vi "Images.vi"() -> ()   [LabVIEW 2019]
uses:
  Classes/Parse/ParseXML/Path.ctl
  Classes/Parse/ParseXML/ParseSVG.lvclass
  Classes/Identity/Identifier.lvclass
  Classes/Identity/Associations.ctl
panel:
  out "String":string
  out "Array 9":string[][](array[string])
  out "Array 2":T1[](array[typedef])
  out "text":string
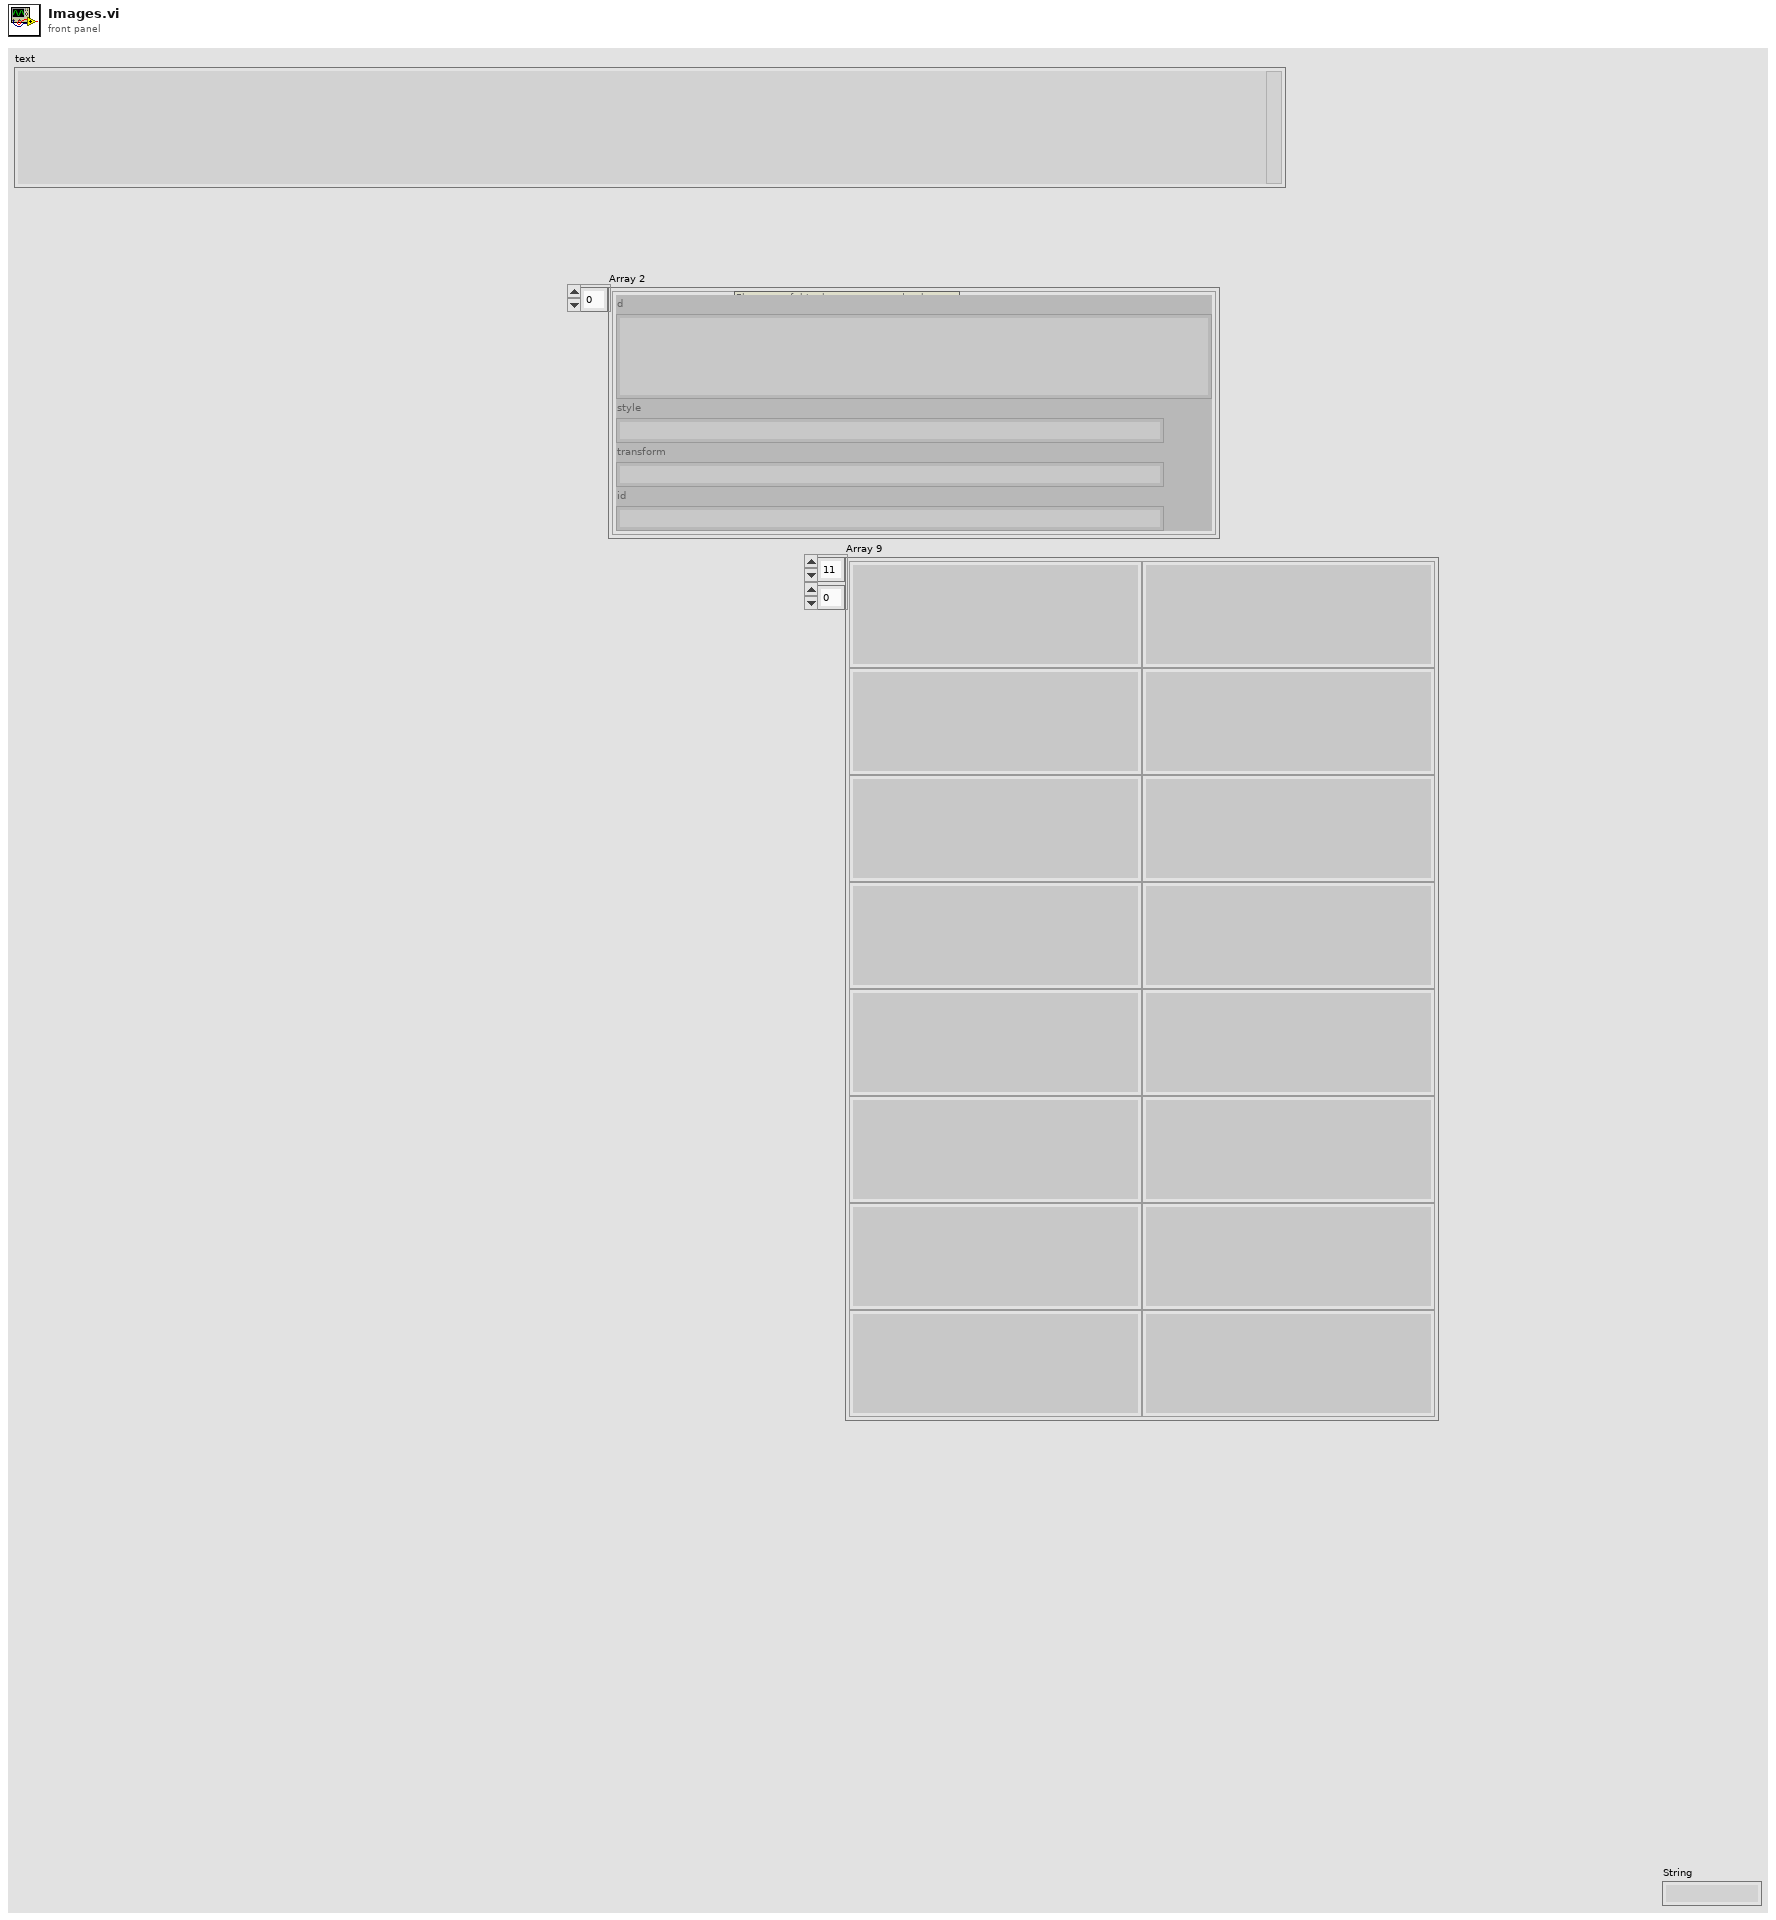
[diagram p1: front panel]
types:
  T1 = typedef "ParseSVG.lvclass/Path.ctl" = cluster{"d":string, "style":string, "transform":string, "id":string}
  T2 = typedef "Identifier.lvclass/Associations.ctl" = cluster{"Name":string, "Alias":string}
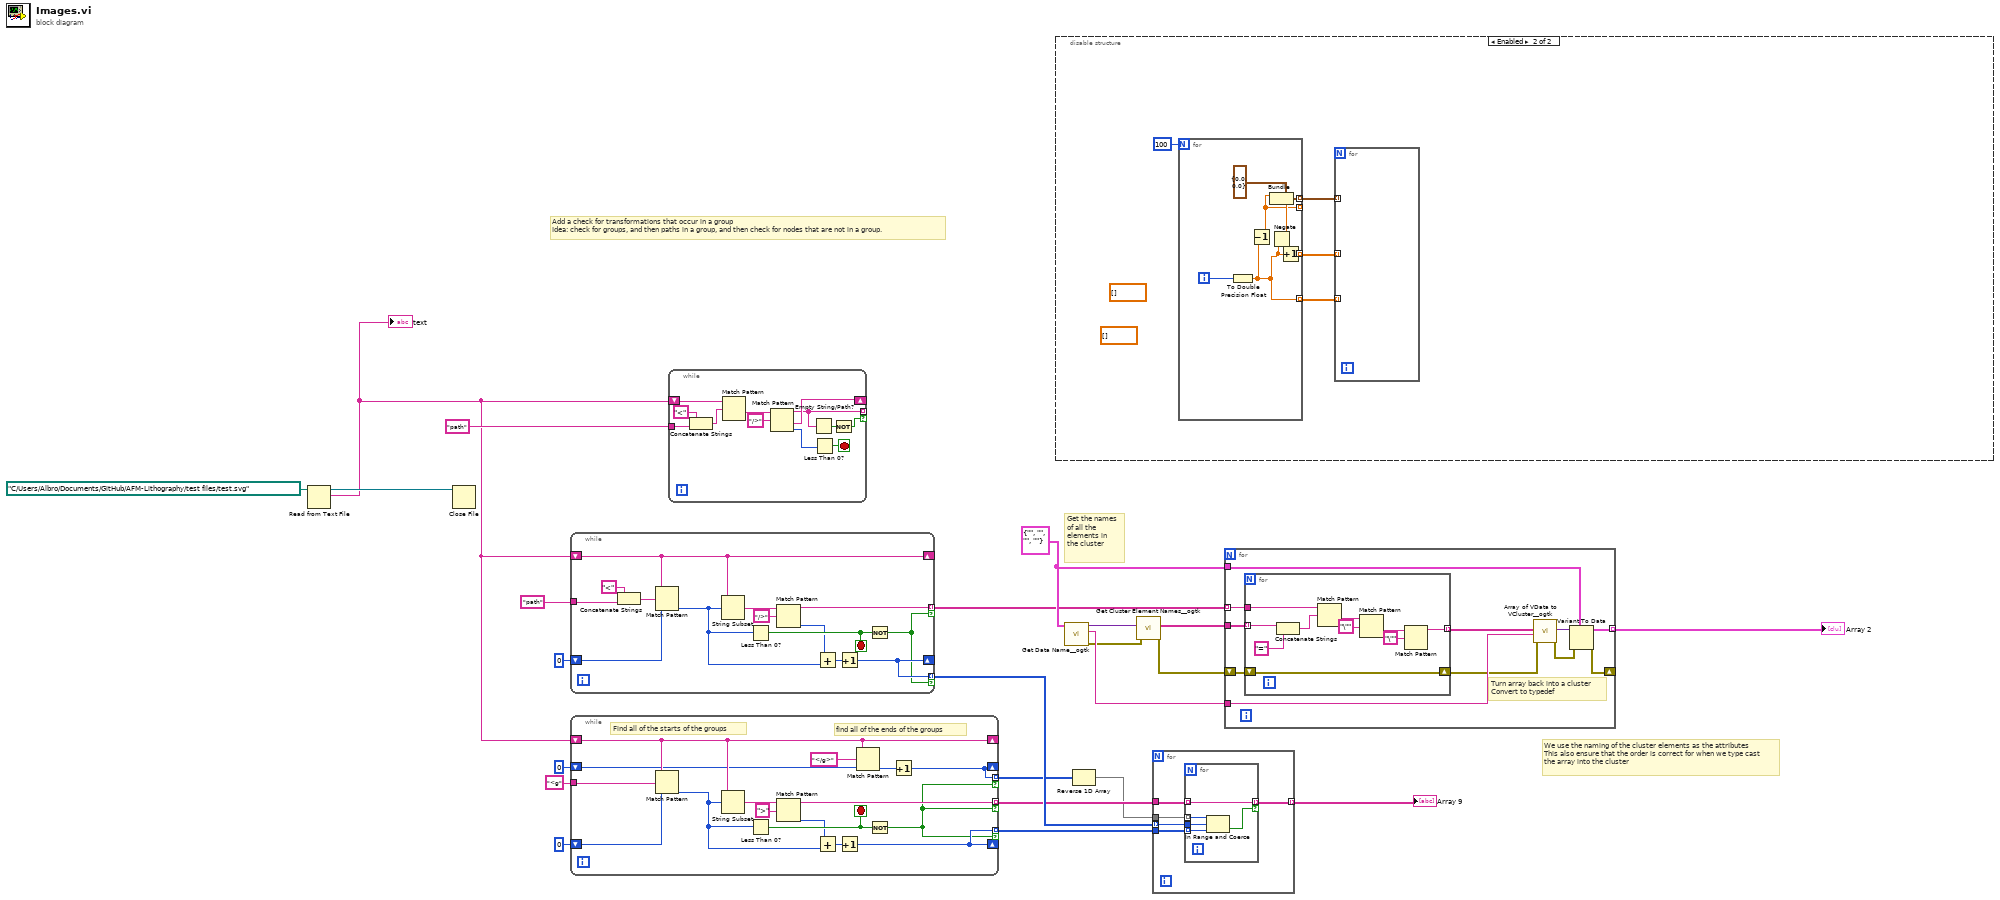
[diagram p0: block diagram]
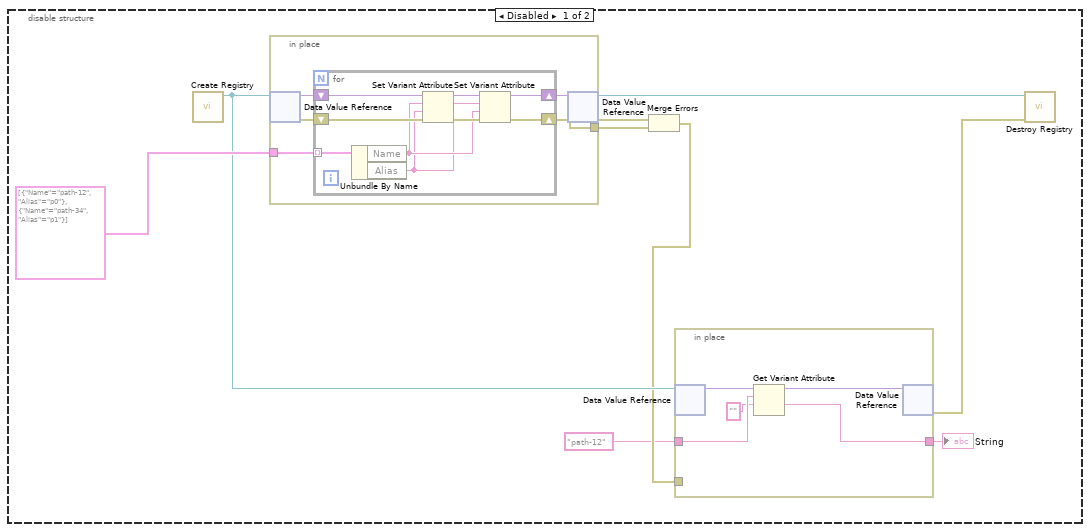
[diagram p2: hidden frame]
diagram:
  w15 = T1 {"d"="", "style"="", "transform"="", "id"=""} ("Path")
  # "Add a check for transformations that occur in a group\nIdea: check for groups, and then paths in a group, and then check for nodes that are not in a group."
  # "We use the naming of the cluster elements as the attributes\nThis also ensure that the order is correct for when we type cast the array into the cluster"
  # "Get the names of all the elements in the cluster"
  n1 = Read from Text File(file (use dialog)=path "C:/Users/Albro/Documents/GitHub/AFM-Lithography/test files/test.svg") -> (refnum out=w23:refnum<file>, text=w3:string)  [unwired: 3 in, 2 out]
  "text" <- w3
  n2 = Close File(refnum=w23) -> ()  [unwired: 1 in, 2 out]
  n3 = while {
    shift-right: [w37] -> _
    shift-left: w3 -> [w37]
    shift-right: [w25] -> _
    shift-left: 0 -> [w35]
    tunnel: [w32] -> w2 mode=indexing if=w24
    tunnel: "path" -> [w26]
    tunnel: [w25] -> w9 mode=indexing if=w24
    stop <- w31 stop-if-true
    n4 = Concatenate Strings("<" ("regular expression"), w26) -> (w28:string)
    n5 = Match Pattern(string=w37, regular expression=w28, offset (0)=w35) -> (offset past match=w29:i32)  [unwired: 3 out]
    n6 = String Subset(string=w37, offset (0)=w29) -> (substring=w36:string)  [unwired: 1 in]
    n7 = Less Than 0?(x=w29) -> (x < 0?=w31:bool)
    n8 = Match Pattern(string=w36, regular expression="/>") -> (before substring=w32:string, offset past match=w30:i32)  [unwired: 1 in, 2 out]
    n9 = Add(x=w30, y=w29) -> (x+y=w34:i32)
    n10 = Increment(x=w34) -> (x+1=w25:i32)
    n11 = Not(x=w31) -> (.not. x?=w24:bool)
  }
  n12 = while {
    shift-right: [w46] -> _
    shift-left: w3 -> [w46]
    shift-right: [w43] -> _
    shift-left: 0 -> [w52]
    tunnel: [w49] -> w7 mode=indexing if=w42
    tunnel: "<g" -> [w38]
    tunnel: [w39] -> w6 mode=indexing if=w42
    tunnel: [w43] -> w8 mode=indexing if=w42
    shift-right: [w39] -> _
    shift-left: 0 ("offset past match") -> [w41]
    stop <- w48 stop-if-true
    # "Find all of the starts of the groups"
    # "find all of the ends of the groups"
    n13 = Match Pattern(string=w46, regular expression=w38, offset (0)=w52) -> (offset past match=w44:i32)  [unwired: 3 out]
    n14 = String Subset(string=w46, offset (0)=w44) -> (substring=w53:string)  [unwired: 1 in]
    n15 = Less Than 0?(x=w44) -> (x < 0?=w48:bool)
    n16 = Match Pattern(string=w53, regular expression=">") -> (before substring=w49:string, offset past match=w47:i32)  [unwired: 1 in, 2 out]
    n17 = Add(x=w47, y=w44) -> (x+y=w51:i32)
    n18 = Increment(x=w51) -> (x+1=w43:i32)
    n19 = Match Pattern(string=w46, regular expression="</g>", offset (0)=w41) -> (offset past match=w40:i32)  [unwired: 3 out]
    n20 = Not(x=w48) -> (.not. x?=w42:bool)
    n21 = Increment(x=w40) -> (x+1=w39:i32)
  }
  n22 = while {
    shift-right: [w58] -> _
    shift-left: w3 -> [w65]
    tunnel: "path" -> [w64]
    tunnel: [w56] -> _ mode=indexing if=w57
    stop <- w60 stop-if-true
    n23 = Concatenate Strings("<" ("regular expression"), w64) -> (w63:string)
    n24 = Match Pattern(string=w65, regular expression=w63) -> (after substring=w62:string)  [unwired: 1 in, 3 out]
    n25 = Match Pattern(string=w62, regular expression="/>") -> (before substring=w56:string, after substring=w58:string, offset past match=w54:i32)  [unwired: 1 in, 1 out]
    n26 = Empty String/Path?(string/path=w56) -> (empty?=w59:bool)
    n27 = Less Than 0?(x=w54) -> (x < 0?=w60:bool)
    n28 = Not(x=w59) -> (.not. x?=w57:bool)
  }
  n29 = disable-structure shown="Enabled" {
    frame Disabled {
      n30 = call "Create Registry.vi"() -> ("Registry"=w70:refnum<data-value>)  [unwired: 10 in, 1 out]
      n31 = in-place {
        in-place-border: [w76] -> w71
        in-place-border: T2[] [{"Name"="path-12", "Alias"="p0"}, {"Name"="path-34", "Alias"="p1"}] -> [w75]
        n32 = in-place-dvr #1(w70) -> (w79:variant, w77:errorcluster)
        n33 = for {
          tunnel: w75 -> [w82] mode=indexing
          shift-right: [w86] -> w78
          shift-left: w79 -> [w88]
          shift-right: [w83] -> w76
          shift-left: w77 -> [w84]
          n34 = Unbundle By Name(w82) -> ("Name"=w81:string, "Alias"=w80:string)
          n35 = Set Variant Attribute(Variant=w88, name=w81, value=w80, error in=w84) -> (Variant out=w87:variant, error out=w85:errorcluster)  [unwired: 1 out]
          n36 = Set Variant Attribute(Variant=w87, name=w80, value=w81, error in=w85) -> (Variant out=w86:variant, error out=w83:errorcluster)  [unwired: 1 out]
        }
        n37 = in-place-dvr #1(w78) -> (w74:refnum<data-value>, w72:errorcluster)
      }
      n38 = Merge Errors(w72, w71) -> (w69:errorcluster)
      n39 = in-place {
        in-place-border: w69 -> [_]
        in-place-border: "path-12" ("name") -> [w91]
        in-place-border: [w89] -> w66
        n40 = in-place-dvr #2(w70) -> (w93:variant)  [unwired: 1 out]
        n41 = Get Variant Attribute(Variant=w93, name=w91, default value (empty Variant)="") -> (duplicate Variant=w92:variant, value=w89:string)  [unwired: 1 in, 2 out]
        n42 = in-place-dvr #2(w92) -> (w68:errorcluster)  [unwired: 1 out]
      }
      "String" <- w66
      n43 = call "Destroy Registry.vi"("error in"=w68, 11:w74) -> ()  [unwired: 9 in, 1 out]
    }
    frame Enabled {
      (unwired) dbl[] [] ("Voltage")
      (unwired) dbl[] [] ("Voltage")
      n44 = for {
        N: 100 -> [_]
        tunnel: [w100] -> w95 mode=indexing
        tunnel: [w103] -> w94 mode=indexing
        tunnel: [w102] -> w96 mode=indexing
        tunnel: [w98] -> _ mode=indexing
        i -> [w104]
        n45 = To Double Precision Float(number=w104) -> (double precision float=w103:dbl)
        n46 = Decrement(x=w103) -> (x-1=w98:dbl)
        n47 = Negate(x=w103) -> (-x=w99:dbl)
        n48 = Bundle(cluster=cluster{"X":dbl, "Y":dbl} {"X"=0.0, "Y"=0.0} ("Point"), "X"=w98, "Y"=w99) -> (w102:cluster{"X":dbl, "Y":dbl})
        n49 = Increment(x=w103) -> (x+1=w100:dbl)
      }
      n50 = for {
        tunnel: w96 -> [_] mode=indexing
        tunnel: w95 -> [_] mode=indexing
        tunnel: w94 -> [_] mode=indexing
      }
    }
  }
  n51 = call <userlib>:"Get Data Name__ogtk.vi"("Data"=w15) -> ("error out"=w16:errorcluster, "Data Name"=w20:string, "Data dup"=w19:variant)  [unwired: 8 in]
  n52 = Reverse 1D Array(array=w6) -> (reversed array=w5:i32[])
  n53 = call <userlib>:"Get Cluster Element Names__ogtk.vi"("error in (no error)"=w16, "Cluster"=w19) -> ("error out"=w17:errorcluster, "Element Names"=w18:string[])  [unwired: 8 in]
  n54 = for {
    tunnel: w9 -> [w109] mode=indexing
    tunnel: w5 -> [w108]
    tunnel: w8 -> [w107]
    tunnel: w7 -> [w106]
    tunnel: [w105] -> w4 mode=indexing
    n55 = for {
      tunnel: w109 -> [w114]
      tunnel: w108 -> [w113] mode=indexing
      tunnel: w107 -> [w112] mode=indexing
      tunnel: w106 -> [w111] mode=indexing
      tunnel: [w111] -> w105 mode=indexing if=w110
      n56 = In Range and Coerce(upper limit=w113, x=w114, lower limit=w112) -> (In Range?=w110:bool)  [unwired: 1 out]
    }
  }
  "Array 9" <- w4
  n57 = for {
    shift-right: [w124] -> _
    shift-left: w17 -> [w123]
    tunnel: [w122] -> w14 mode=indexing
    tunnel: w18 -> [w119]
    tunnel: w20 -> [w118]
    tunnel: w15 -> [w117]
    tunnel: w2 -> [w115] mode=indexing
    # "Turn array back into a cluster\nConvert to typedef"
    n58 = for {
      shift-right: [w135] -> w116
      shift-left: w123 -> [w135]
      tunnel: [w129] -> w121 mode=indexing
      tunnel: w119 -> [w127] mode=indexing
      tunnel: w115 -> [w134]
      n59 = Concatenate Strings(w127, "=" ("string")) -> (w128:string)
      n60 = Match Pattern(string=w134, regular expression=w128) -> (after substring=w133:string)  [unwired: 1 in, 3 out]
      n61 = Match Pattern(string=w133, regular expression="\"") -> (after substring=w131:string)  [unwired: 1 in, 3 out]
      n62 = Match Pattern(string=w131, regular expression="\"") -> (before substring=w129:string)  [unwired: 1 in, 3 out]
    }
    n63 = call <userlib>:"Array of VData to VCluster__ogtk.vi"("error in (no error)"=w116, "Cluster Name"=w118, "Array"=w121) -> ("error out"=w125:errorcluster, "VCluster"=w120:variant)  [unwired: 7 in]
    n64 = Variant To Data(error in=w125, type=w117, Variant=w120) -> (data=w122:T1, error out=w124:errorcluster)
  }
  "Array 2" <- w14
